vi "GetSetTrigger.vi"(7 "Set":bool, 8 "error in (no error)":errorcluster, 10 "Source":string, 11 "Camera in":refnum<class "Camera.lvclass">) -> (0 "error out":errorcluster, 3 "Source":string)   [LabVIEW 2020, in "Camera.lvclass"]
uses:
  Camera.lvclass
  Camera.lvclass/Camera.ctl
  bin/gindustrialcam_32-1.dll
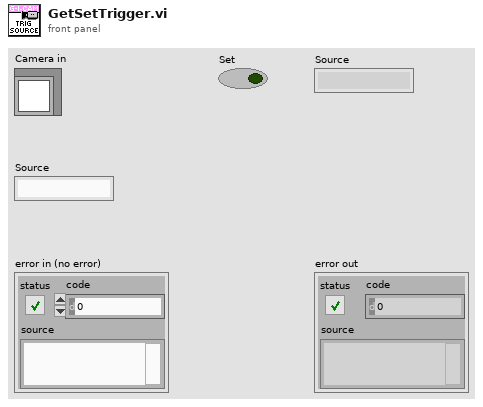
[diagram p1: front panel]
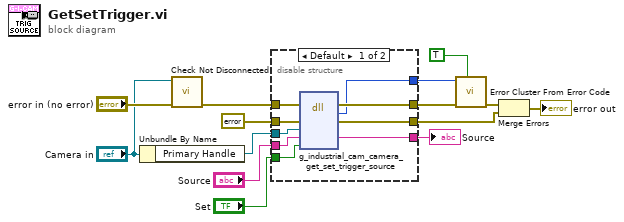
[diagram p0: block diagram]
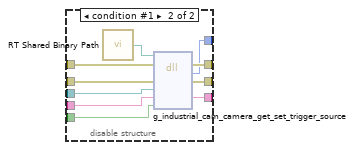
[diagram p2: hidden frame]
diagram:
  n1 = Unbundle By Name("Camera in") -> ("Primary Handle"=w2:refnum<data-value>)
  n2 = call "Check Not Disconnected.vi"("error in (no error)"="error in (no error)", "Camera in"="Camera in") -> ("error out"=w3:errorcluster)  [unwired: 9 in]
  n3 = disable-structure shown="Default" {
    disable-tunnel: "Set" -> [w23 w33]
    disable-tunnel: [w22 w32] -> w13
    disable-tunnel: [w21 w31] -> w12
    disable-tunnel: [w20 w30] -> w10
    disable-tunnel: errorcluster {"status"=FALSE, "code"=0, "source"=""} ("error constant") -> [w19 w29]
    disable-tunnel: "Source" -> [w18 w28]
    disable-tunnel: [w17 w27] -> w4
    disable-tunnel: w3 -> [w16 w26]
    disable-tunnel: w2 -> [w15 w25]
    frame condition #0 (active) {
      n4 = dll-call lib="C:/serenial/lib/g-industrial-camera/LabVIEW/g_industrial_cam/bin/gindustrialcam_*-1.*" fn="g_industrial_cam_camera_get_set_trigger_source"(error in=w16, "err"=w19, "edvr"=w15, "formats"=w18, "set"=w23) -> (error out=w22:errorcluster, "Mg_Error"=w21:i32, "err"=w20:errorcluster, "formats"=w17:string)  [unwired: 4 in, 1 out]
    }
    frame condition #1 {
      n5 = call "RT Shared Binary Path.vi"() -> ("Path"=w24:path)
      n6 = dll-call lib="C:/serenial/lib/g-industrial-camera/LabVIEW/g_industrial_cam/bin/gindustrialcam_*-1.*" fn="g_industrial_cam_camera_get_set_trigger_source"(path in=w24, error in=w26, "err"=w29, "edvr"=w25, "formats"=w28, "set"=w33) -> (error out=w32:errorcluster, "Mg_Error"=w31:i32, "err"=w30:errorcluster, "formats"=w27:string)  [unwired: 3 in, 1 out]
    }
  }
  "Source" <- w4
  n7 = call <vilib>:"Error Cluster From Error Code.vi"("show call chain? (False)"=TRUE, "error in (no error)"=w13, "error code (0)"=w12) -> ("error out"=w11:errorcluster)  [unwired: 6 in]
  n8 = Merge Errors(w11, w10) -> (→"error out":errorcluster)
